vi "hand_inference_v001.vi"() -> ()   [LabVIEW 2025]
uses:
  <vilib>/Utility/error.llb/Trim Whitespace One-Sided.vi
  <vilib>/MakerHub/Leap/LMH-Leap.lvlib
panel:
  out "Common.Duration (S)":dbl
  in  "Slide":dbl(slide) scale=0.0..10.0
  out "Direction.Magnitude":sgl
  out "element":sgl
  out "String":string
  out "Current Word":string
  out "Current Letter":string
  out "Output":string
  in  "?":bool
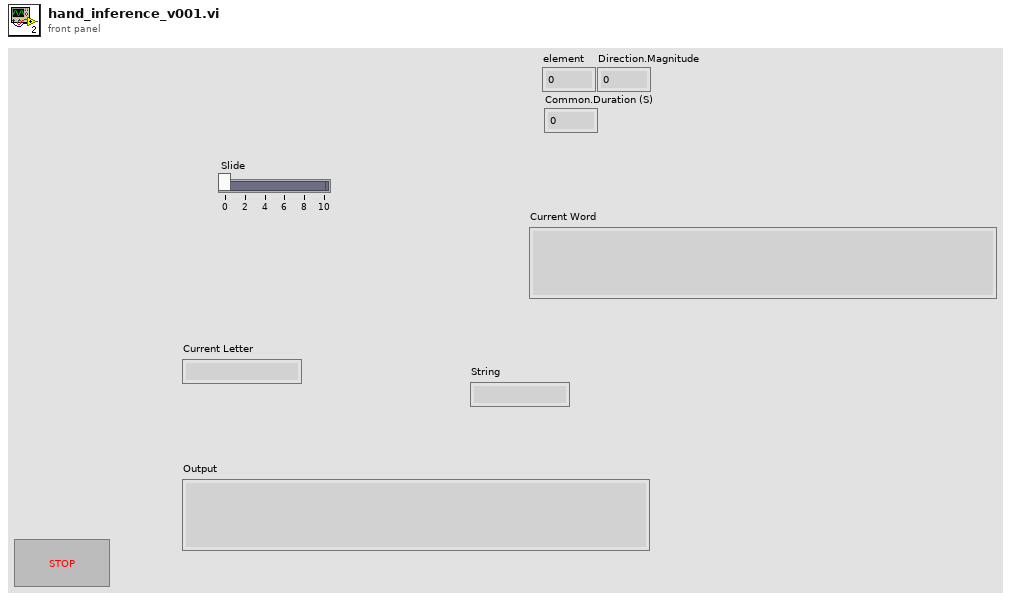
[diagram p1: front panel]
types:
  T1 = typedef "LMH-Leap.lvlib/Leap Handle.ctl" = cluster{"LeapCSharp":refnum<k24>}
  T2 = typedef "LMH-Leap.lvlib/Frame.ctl" = cluster{"ID":i64, "Timestamp":i64, "Current FPS":dbl, "Key Tap Gestures":T3[], "Circle Gestures":T8[], "Screen Tap Gestures":T9[], "Swipe Gestures":T10[], "Hands":T11[]}
  T3 = typedef "LMH-Leap.lvlib/Gesture Key Tap.ctl" = cluster{"Common":T4, "Direction":T7, "Position":T7, "Progress":dbl}
  T4 = typedef "LMH-Leap.lvlib/Gesture Common.ctl" = cluster{"ID":dbl, "Duration (S)":dbl, "Gesture Type":T5, "Gesture State":T6}
  T5 = typedef "LMH-Leap.lvlib/Gesture Type.ctl" = enum16{"Invalid", "Swipe", "Circle", "Screen Tap", "Key Tap"}
  T6 = typedef "LMH-Leap.lvlib/Gesture State.ctl" = enum16{"Invalid", "Start", "Update", "Stop"}
  T7 = typedef "LMH-Leap.lvlib/Vector.ctl" = cluster{"Pitch":sgl, "Yaw":sgl, "Roll":sgl, "Magnitude":sgl, "XYZ":sgl[]}
  T8 = typedef "LMH-Leap.lvlib/Gesture Circle.ctl" = cluster{"Common":T4, "Center":T7, "Normal":T7, "Progress":dbl, "Radius":dbl}
  T9 = typedef "LMH-Leap.lvlib/Gesture Screen Tap.ctl" = cluster{"Common":T4, "Direction":T7, "Position":T7, "Progress":dbl}
  T10 = typedef "LMH-Leap.lvlib/Gesture Swipe.ctl" = cluster{"Common":T4, "Direction":T7, "Position":T7, "Start Position":T7, "Speed":dbl}
  T11 = typedef "LMH-Leap.lvlib/Hand.ctl" = cluster{"Palm Normal":T7, "Palm Position":T7, "Palm Velocity":T7, "Direction":T7, "Palm Position (Stabilized)":T7, "Sphere Center":T7, "Pointables":T12[], "ID":i32, "Time Visible":sgl, "Sphere Radius":sgl}
  T12 = typedef "LMH-Leap.lvlib/Pointable.ctl" = cluster{"Type":T13, "Touch Zone":T14, "ID":i32, "Length":dbl, "Width":dbl, "Time Visible":dbl, "Touch Distance":dbl, "Direction":T7, "Tip Position":T7, "Tip Velocity":T7, "Tip Position (Stabilized)":T7}
  T13 = typedef "LMH-Leap.lvlib/Pointable Type.ctl" = enum16{"Finger", "Tool"}
  T14 = typedef "LMH-Leap.lvlib/Pointable Zone.ctl" = enum16{"None", "Hovering", "Touching"}
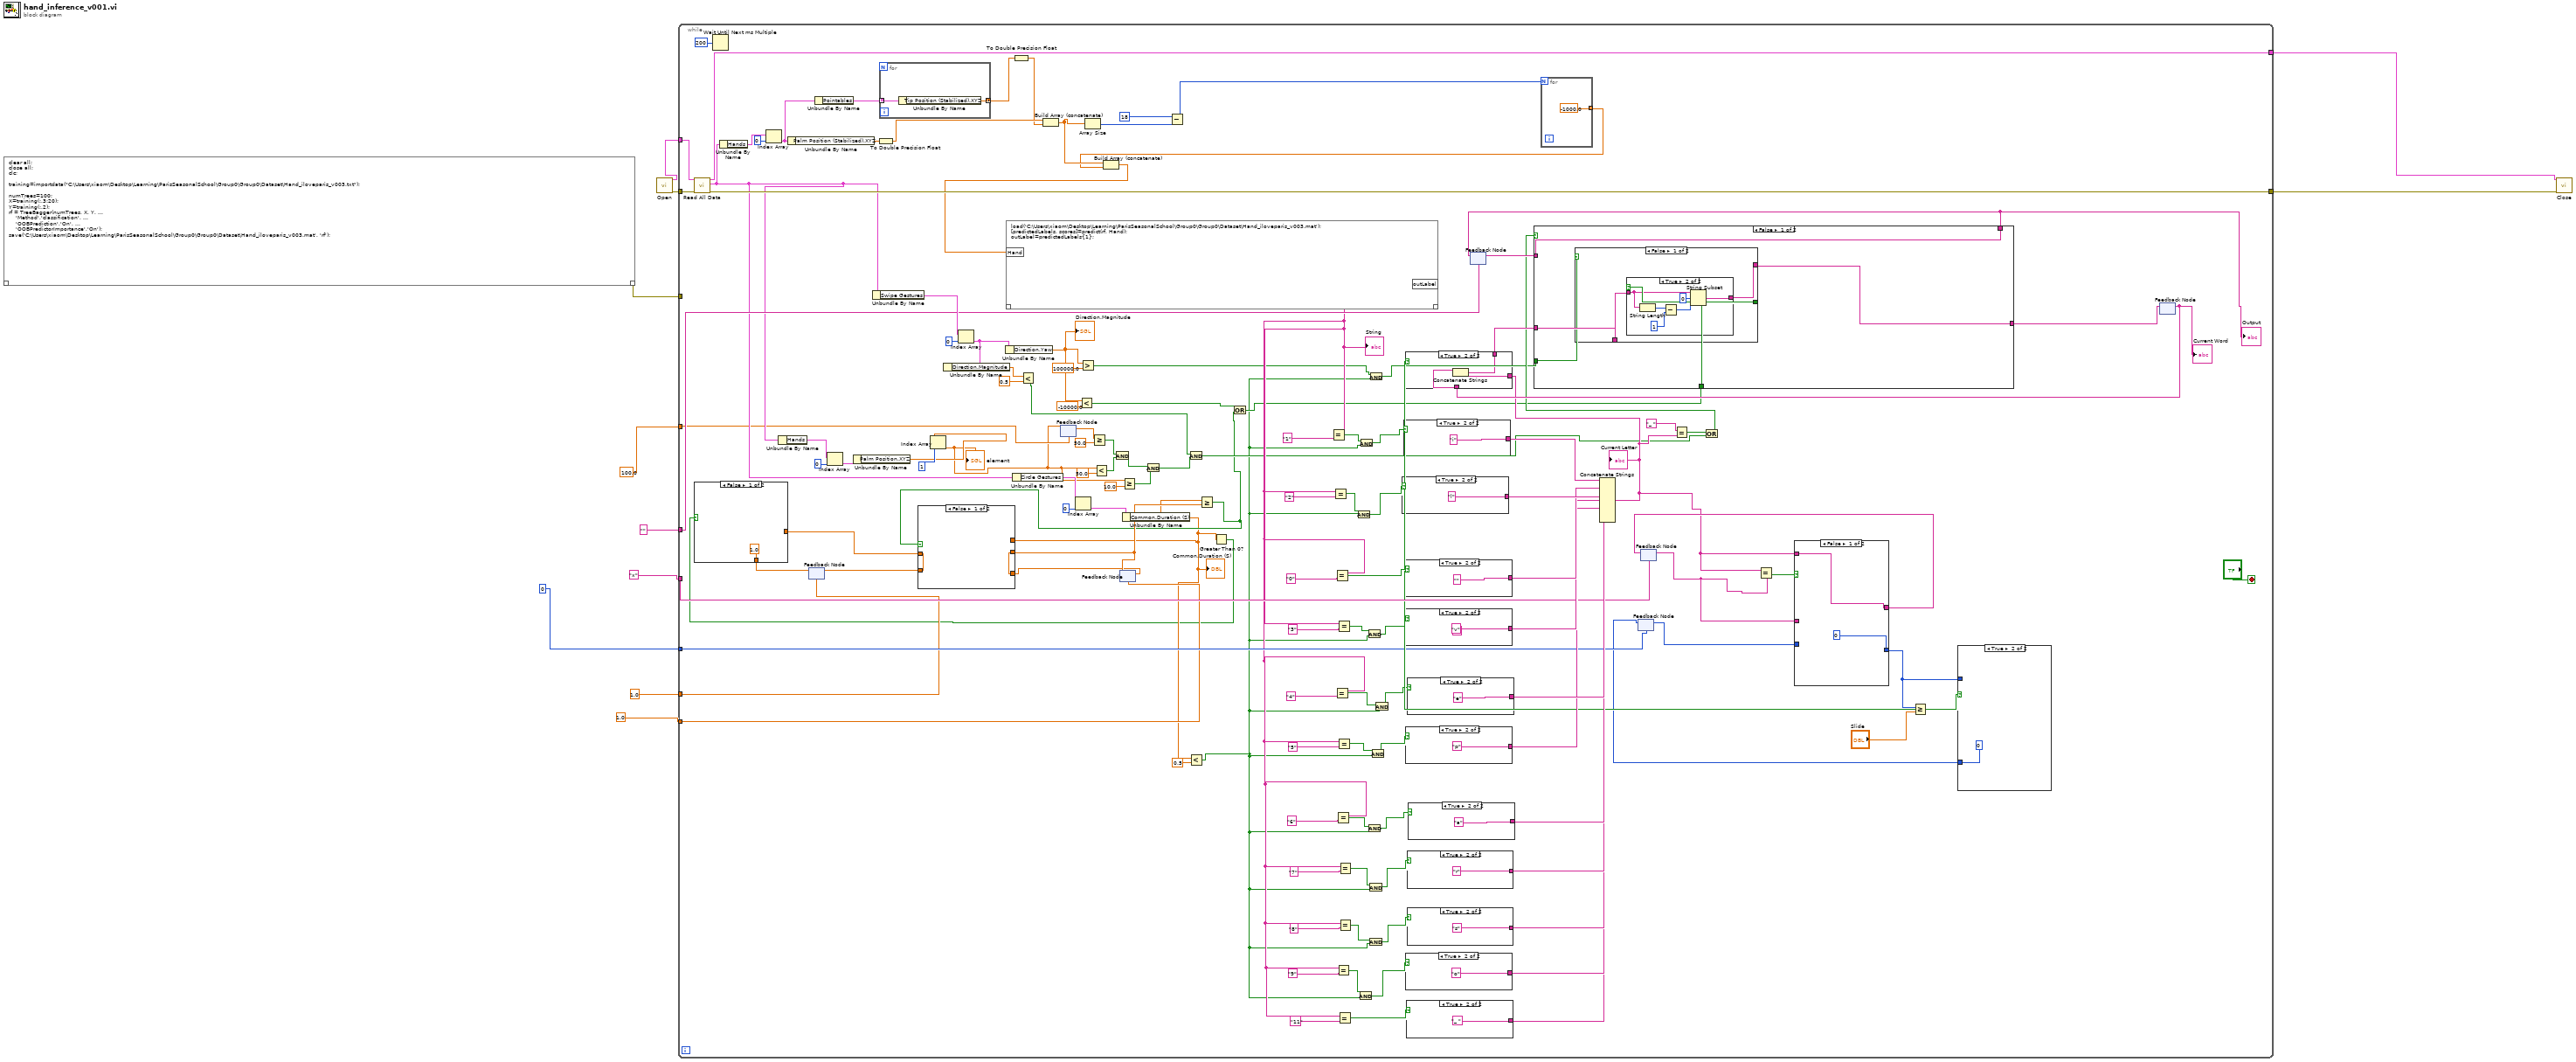
[diagram p0: block diagram]
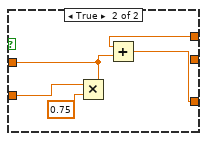
[diagram p3: hidden frame]
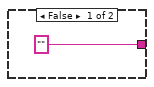
[diagram p4: hidden frame]
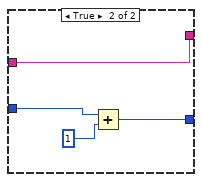
[diagram p6: hidden frame]
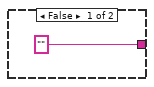
[diagram p7: hidden frame]
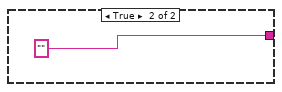
[diagram p10: hidden frame]
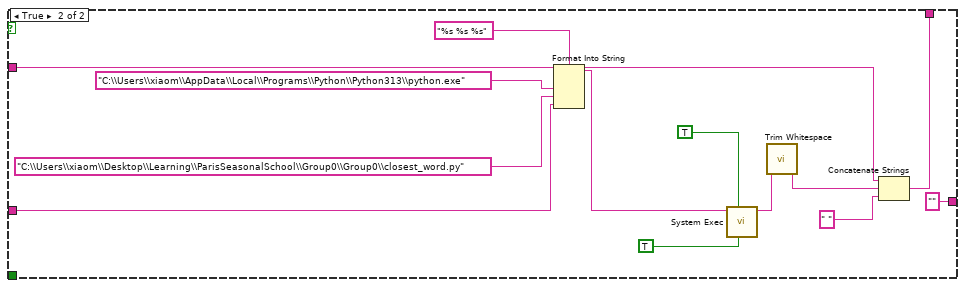
[diagram p11: hidden frame]
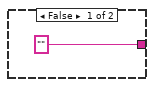
[diagram p12: hidden frame]
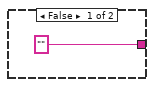
[diagram p13: hidden frame]
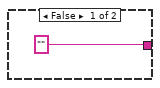
[diagram p14: hidden frame]
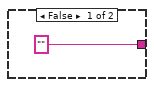
[diagram p15: hidden frame]
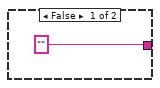
[diagram p16: hidden frame]
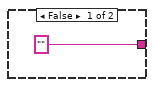
[diagram p17: hidden frame]
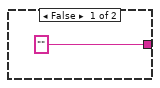
[diagram p18: hidden frame]
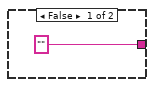
[diagram p19: hidden frame]
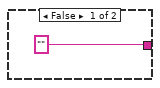
[diagram p20: hidden frame]
diagram:
  n1 = script code="clear all;\nclose all;\nclc;\n\ntraining=importdata(\"C:\\Users\\xiaom\\Desktop\\Learning\\ParisSeasonalSchool\\Group0\\Group0\\Dataset\\Hand_iloveparis_v003.txt\");\n\nnumTrees=100;\nX=training(:,3:20);\nY=training(:,2);\nrf = TreeBagger(numTrees, X, Y, ...\n    'Method','classification', ...\n    'OOBPrediction','On', ...\n    'OOBPredictorImportance','On');\nsave('C:\\Users\\xiaom\\Desktop\\Learning\\ParisSeasonalSchool\\Group0\\Group0\\Dataset\\Hand_iloveparis_v003.mat', 'rf');"() -> ("??"=w7:errorcluster)  [unwired: 1 in]
  n2 = call <vilib>:"Open.vi"() -> ("Error Out"=w10:errorcluster, "Leap Handle"=w11:T1)  [unwired: 10 in]
  n3 = while {
    tunnel: w11 -> [w140]
    tunnel: w10 -> [w139]
    tunnel: [w138] -> w9
    tunnel: [w137] -> w8
    tunnel: w7 -> [_]
    tunnel: "x" -> [w92]
    tunnel: 0 -> [w88]
    tunnel: "" -> [w80]
    tunnel: 100.0 -> [w64]
    tunnel: 1.0 -> [w45]
    tunnel: 1.0 -> [w17]
    stop <- "?" stop-if-true
    n4 = call <vilib>:"Read All Data.vi"("Error In"=w139, "Leap Handle"=w140) -> ("Error Out"=w137:errorcluster, "Frame"=w71:T2, "Leap Handle"=w138:T1)  [unwired: 6 in, 1 out]
    n5 = Wait Until Next ms Multiple(millisecond multiple=u32 200) -> ()  [unwired: 1 out]
    n6 = Unbundle By Name(w71) -> ("Hands"=w134:T11[])
    n7 = Index Array(array=w134, index=0) -> (element=w98:T11)
    n8 = Unbundle By Name(w71) -> ("Hands"=w69:T11[])
    n9 = Unbundle By Name(w98) -> ("Palm Position (Stabilized).XYZ"=w132:sgl[])
    n10 = feedback #1(w17) -> (w16:dbl)
    n11 = Unbundle By Name(w98) -> ("Pointables"=w128:T12[])
    n12 = Index Array(array=w69, index=0) -> (element=w68:T11)
    n13 = Unbundle By Name(w68) -> ("Palm Position.XYZ"=w66:sgl[])
    n14 = Unbundle By Name(w71) -> ("Swipe Gestures"=w97:T10[])
    n15 = To Double Precision Float(number=w132) -> (double precision float=w130:dbl[])
    n16 = for {
      tunnel: w128 -> [w215] mode=indexing
      tunnel: [w214] -> w131 mode=concatenating
      n17 = Unbundle By Name(w215) -> ("Tip Position (Stabilized).XYZ"=w214:sgl[])
    }
    n18 = Index Array(array=w66, index=1) -> (element=w54:sgl)
    "element" <- w54
    n19 = Index Array(array=w97, index=0) -> (element=w50:T10)
    n20 = Unbundle By Name(w50) -> ("Direction.Magnitude"=w48:sgl)
    n21 = Unbundle By Name(w50) -> ("Direction.Yaw"=w94:sgl)
    "Direction.Magnitude" <- w94
    n22 = Unbundle By Name(w71) -> ("Circle Gestures"=w81:T8[])
    n23 = To Double Precision Float(number=w131) -> (double precision float=w129:dbl[])
    n24 = Less?(x=w48, y=sgl 0.5) -> (x < y?=w49:bool)
    n25 = Build Array (concatenate)(w130, w129) -> (w124:dbl[])
    n26 = feedback #2(w64) -> (w63:dbl)
    n27 = feedback-in #2(w54) -> ()
    n28 = Index Array(array=w81, index=0) -> (element=w83:T8)
    n29 = Less?(x=w94, y=sgl -10000.0) -> (x < y?=w42:bool)
    n30 = Greater?(x=w94, y=sgl 100000.0) -> (0:w39:bool)
    n31 = Array Size(array=w124) -> (size(s)=w127:i32)
    n32 = Greater Or Equal?(x=w63, y=50.0) -> (x >= y?=w59:bool)
    n33 = Less?(x=w54, y=sgl 50.0) -> (x < y?=w60:bool)
    n34 = And(x=w59, y=w60) -> (x .and. y?=w55:bool)
    n35 = feedback #3(w45) -> (w44:dbl)
    n36 = Greater Or Equal?(x=w54, y=sgl 10.0) -> (x >= y?=w56:bool)
    n37 = Unbundle By Name(w83) -> ("Common.Duration (S)"=w13:dbl)
    "Common.Duration (S)" <- w13
    n38 = And(x=w55, y=w56) -> (x .and. y?=w51:bool)
    n39 = Subtract(x=18, y=w127) -> (x-y=w125:i32)
    n40 = And(x=w49, y=w51) -> (x .and. y?=w52:bool)
    n41 = Less?(x=w13, y=0.5) -> (x < y?=w19:bool)
    n42 = Greater Or Equal?(x=w13, y=w44) -> (x >= y?=w18:bool)
    n43 = case shown="False" w18 {
      tunnel: [w144 w148] -> w43
      tunnel: w44 -> [w144 _]
      tunnel: w13 -> [_ w149]
      tunnel: w16 -> [w143 w147]
      tunnel: [w143 w145] -> w15
      frame False {
      }
      frame True {
        n44 = Multiply(x=w147, y=0.75) -> (x*y=w145:dbl)
        n45 = Add(x=w149, y=w145) -> (x+y=w148:dbl)
      }
    }
    n46 = feedback-in #3(w43) -> ()
    n47 = Greater Than 0?(x=w13) -> (x > 0?=w12:bool)
    n48 = case shown="False" w12 {
      tunnel: w15 -> [_ w142]
      tunnel: [1.0 w142] -> w14
      frame False {
      }
      frame True {
      }
    }
    n49 = feedback-in #1(w14) -> ()
    n50 = Or(x=w42, y=w18) -> (x .or. y?=w41:bool)
    n51 = And(x=w39, y=w19) -> (x .and. y?=w38:bool)
    n52 = feedback #4(w80) -> (w79:string)
    n53 = for {
      N: w125 -> [_]
      tunnel: [-1000.0] -> w123 mode=indexing
    }
    n54 = Build Array (concatenate)(w124, w123) -> (w122:dbl[])
    n55 = script code="load('C:\\Users\\xiaom\\Desktop\\Learning\\ParisSeasonalSchool\\Group0\\Group0\\Dataset\\Hand_iloveparis_v003.mat');\n[predictedLabels, scores]=predict(rf, Hand);\noutLabel=predictedLabels{1};"("Hand"=w122) -> ("outLabel"=w65:string)  [unwired: 1 in, 1 out]
    "String" <- w65
    n56 = Equal?(x=w65, y="1") -> (x = y?=w37:bool)
    n57 = Equal?(x=w65, y="2") -> (x = y?=w35:bool)
    n58 = Equal?(x=w65, y="0") -> (x = y?=w118:bool)
    n59 = Equal?(x=w65, y="4") -> (x = y?=w31:bool)
    n60 = Equal?(x=w65, y="6") -> (x = y?=w21:bool)
    n61 = Equal?(x=w65, y="9") -> (x = y?=w27:bool)
    n62 = Equal?(x=w65, y="3") -> (x = y?=w33:bool)
    n63 = Equal?(x=w65, y="5") -> (x = y?=w29:bool)
    n64 = Equal?(x=w65, y="11") -> (x = y?=w76:bool)
    n65 = Equal?(x=w65, y="7") -> (x = y?=w23:bool)
    n66 = Equal?(x=w65, y="8") -> (x = y?=w25:bool)
    n67 = And(x=w35, y=w19) -> (x .and. y?=w34:bool)
    n68 = And(x=w27, y=w19) -> (x .and. y?=w26:bool)
    n69 = And(x=w37, y=w19) -> (x .and. y?=w36:bool)
    n70 = And(x=w33, y=w19) -> (x .and. y?=w32:bool)
    n71 = And(x=w21, y=w19) -> (x .and. y?=w20:bool)
    n72 = And(x=w23, y=w19) -> (x .and. y?=w22:bool)
    n73 = And(x=w25, y=w19) -> (x .and. y?=w24:bool)
    n74 = And(x=w29, y=w19) -> (x .and. y?=w28:bool)
    n75 = And(x=w31, y=w19) -> (x .and. y?=w30:bool)
    n76 = case shown="True" w34 {
      tunnel: ["" "l"] -> w110
      frame False {
      }
      frame True {
      }
    }
    n77 = case shown="True" w36 {
      tunnel: ["" "i"] -> w119
      frame False {
      }
      frame True {
      }
    }
    n78 = case shown="True" w26 {
      tunnel: ["" "o"] -> w99
      frame False {
      }
      frame True {
      }
    }
    n79 = case shown="True" w118 {
      tunnel: ["" ""] -> w109
      frame False {
      }
      frame True {
      }
    }
    n80 = case shown="True" w32 {
      tunnel: ["" "v"] -> w108
      frame False {
      }
      frame True {
        (unwired) "v"
      }
    }
    n81 = case shown="True" w28 {
      tunnel: ["" "p"] -> w106
      frame False {
      }
      frame True {
      }
    }
    n82 = case shown="True" w76 {
      tunnel: ["" "_ "] -> w74
      frame False {
      }
      frame True {
      }
    }
    n83 = case shown="True" w22 {
      tunnel: ["" "r"] -> w104
      frame False {
      }
      frame True {
      }
    }
    n84 = case shown="True" w24 {
      tunnel: ["" "s"] -> w103
      frame False {
      }
      frame True {
      }
    }
    n85 = case shown="True" w30 {
      tunnel: ["" "e"] -> w107
      frame False {
      }
      frame True {
      }
    }
    n86 = case shown="True" w20 {
      tunnel: ["" "a"] -> w105
      frame False {
      }
      frame True {
      }
    }
    n87 = Concatenate Strings(w119, w110, w109, w105, w103, w108, w107, w106, w104, w99, w74) -> (w73:string)
    "Current Letter" <- w73
    n88 = feedback #5(w88) -> (w87:i32)
    n89 = feedback #6(w92) -> (w90:string)
    n90 = Equal?(x="_ ", y=w73) -> (x = y?=w58:bool)
    n91 = Or(x=w58, y=w52) -> (x .or. y?=w57:bool)
    n92 = Equal?(x=w73, y=w90) -> (x = y?=w89:bool)
    n93 = case shown="False" w89 {
      tunnel: w90 -> [_ w156]
      tunnel: w73 -> [w155 _]
      tunnel: [w155 w156] -> w84
      tunnel: w87 -> [_ w159]
      tunnel: [0 ("y") w157] -> w85
      frame False {
      }
      frame True {
        n94 = Add(x=w159, y=1) -> (x+y=w157:i32)
      }
    }
    n95 = feedback-in #6(w84) -> ()
    n96 = Greater Or Equal?(x=w85, y="Slide") -> (x >= y?=w91:bool)
    n97 = case shown="True" w91 {
      tunnel: [w152 0 ("y")] -> w86
      tunnel: w85 -> [w152 _]
      frame False {
      }
      frame True {
      }
    }
    n98 = feedback-in #5(w86) -> ()
    n99 = feedback #7() -> (w77:string)  [unwired: 1 in]
    "Current Word" <- w77
    n100 = case shown="True" w91 {
      tunnel: w73 -> [_ w163]
      tunnel: w77 -> [w162 w164]
      tunnel: [w162 w165] -> w102
      frame False {
      }
      frame True {
        n101 = Concatenate Strings(w164, w163) -> (w165:string)
      }
    }
    n102 = case shown="False" w57 {
      tunnel: [w169 ""] -> w101
      tunnel: w102 -> [w170 w188]
      tunnel: w38 -> [w168 _]
      tunnel: w41 -> [w167 _]
      tunnel: w79 -> [w166 w184]
      tunnel: [w166 w183] -> w78
      frame False {
        n103 = case shown="False" w168 {
          tunnel: [w171 ""] -> w169
          tunnel: w170 -> [w172 _]
          tunnel: w167 -> [w173 _]
          frame False {
            n104 = case shown="True" w173 {
              tunnel: [w174 w180] -> w171
              tunnel: w172 -> [w174 w178]
              frame False {
              }
              frame True {
                n105 = String Length(string=w178) -> (length=w176:i32)
                n106 = Subtract(x=w176, y=1 ("offset (0)")) -> (x-y=w175:i32)
                n107 = String Subset(string=w178, offset (0)=0, length (rest)=w175) -> (substring=w180:string)
              }
            }
          }
          frame True {
          }
        }
      }
      frame True {
        n108 = Format Into String(format string="%s %s %s", "C:\\Users\\xiaom\\AppData\\Local\\Programs\\Python\\Python313\\python.exe" ("input 6"), "C:\\Users\\xiaom\\Desktop\\Learning\\ParisSeasonalSchool\\Group0\\Group0\\closest_word.py" ("input 6"), w188) -> (resulting string=w191:string)  [unwired: 2 in, 1 out]
        n109 = call <vilib>:"System Exec.vi"("run minimized? (F)"=TRUE, "wait until completion? (T)"=TRUE, "command line"=w191) -> ("standard output"=w187:string)  [unwired: 5 in, 3 out]
        n110 = call <vilib>:"Trim Whitespace.vi"("string"=w187) -> ("trimmed string"=w185:string)  [unwired: 1 in]
        n111 = Concatenate Strings(w184, w185, " ") -> (w183:string)
      }
    }
    "Output" <- w78
    n112 = feedback-in #4(w78) -> ()
    n113 = feedback-in #7(w101) -> ()
  }
  n114 = call <vilib>:"Close.vi"("Error In"=w8, "Leap Handle"=w9) -> ()  [unwired: 9 in, 1 out]
